vi "DMA Channel.vi"(8 "error in (no error)":errorcluster, 11 "Node Ptr":T3 format="%.0x") -> (0 "error out":errorcluster)   [LabVIEW 2020, in "FPGA Addon System Explorer.lvlib"]
uses:
  FPGA Addon System Explorer.lvlib
  <vilib>/NI VeriStand/Custom Device API/Custom Device API.lvlib
  Addon Shared/FPGA Addon Shared.lvlib
  Addon Shared/Types/FG Action.ctl
  Addon Shared/Types/Delacing Scheme.ctl
  Addon Shared/Types/DMA Acquisition Mode.ctl
  Addon Shared/Types/DMA Settings.ctl
  <vilib>/NI VeriStand/Custom Device API/Custom Device Item Ref.ctl
panel:
  in  "DMA Host Buffer":u32(ring)=5 items=["1 Second"=1, "2 Seconds"=2, "5 Seconds"=5, "10 Seconds"=10]
  out "Original Name":string
  in  "Number of Samples":u32
  in  "Mode":T1
  in  "dt":dbl format="%#_p"
  in  "Reset":bool
  in  "Apply":bool
  in  "Update Rate":u32(ring)=1 items=["1 Hz"=1, "2 Hz"=2, "5 Hz"=5, "10 Hz"=10]
  in  "Delacing Scheme":T2
  in  "Number of Channels":u8
  in  "Header 2":cluster{"Section Name":string}={"Section Name"="DMA Settings"}
  in  "SHDocVw.IWebBrowser":refnum<k7>(container)
  in  "Header":cluster{"Section Name":string}={"Section Name"="Section Settings"}
  in  "Description":string
  in  "Name":string
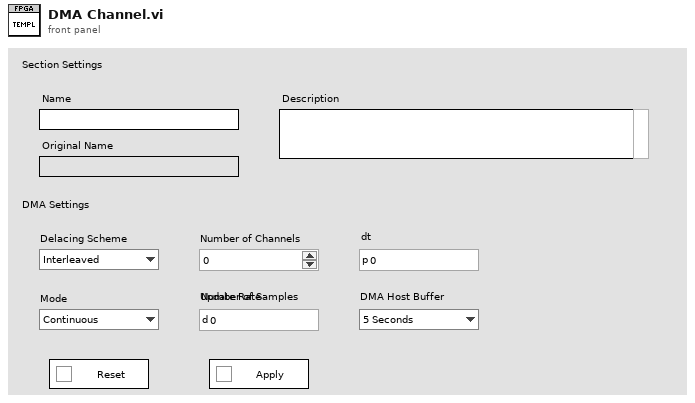
[diagram p1: front panel]
types:
  T1 = typedef "FPGA Addon Shared.lvlib/DMA Acquisition Mode.ctl" = enum8{"Continuous", "Triggered Finite"}
  T2 = typedef "FPGA Addon Shared.lvlib/Delacing Scheme.ctl" = enum8{"Interleaved", "Bitpacked"}
  T3 = typedef "Custom Device API.lvlib/Custom Device Item Ref.ctl" = u64
  T4 = typedef "FPGA Addon Shared.lvlib/FG Action.ctl" = enum8{"GET", "SET"}
  T5 = typedef "FPGA Addon Shared.lvlib/DMA Information.ctl" = cluster{"Name":string, "Data Type":T6}
  T6 = typedef "FPGA Addon Shared.lvlib/FPGA Addon Data Type.ctl" = enum8{"<Null>", "I8", "I16", "I32", "I64", "U8", "U16", "U32", "U64", "SGL", "Boolean", "Analog PWM In Settings", "Analog PWM In", "Digital PWM In Settings", "Digital PWM In", "Digital PWM Out", "Sine Out", "FXP", "FXP+/-24.5", "FXP+/-16.5", "FXP+/-32.8", "FXP+/-64.32", "FXP+/-16.7", "FXP+/-20.5", "FXP+/-27.5", "FXP+/-32.16", "FXP+16.3", "FXP+18.3", "Digital Static In", "Digital Static Out", "Digital Static In Settings", "Digital WSS Out", "Quad Encoder Settings", "Quad Encoder In", "Group"}
  T7 = typedef "Custom Device API.lvlib/Custom Device Item Info.ctl" = cluster{"Name":string, "Is Channel":bool, "GUID":string, "Is Waveform":bool}
  T8 = typedef "FPGA Addon Shared.lvlib/DMA Settings.ctl" = cluster{"Number of Channels":u8, "Delacing Scheme":T2, "Update Rate":u32, "dt":dbl, "Mode":T1, "Number of Samples":u32, "DMA Host Buffer":u32}
  T9 = typedef "Custom Device API.lvlib/Custom Device Commands.ctl" = enum16{"Default", "Item renamed", "Shutdown", "Dynamic button pressed"}
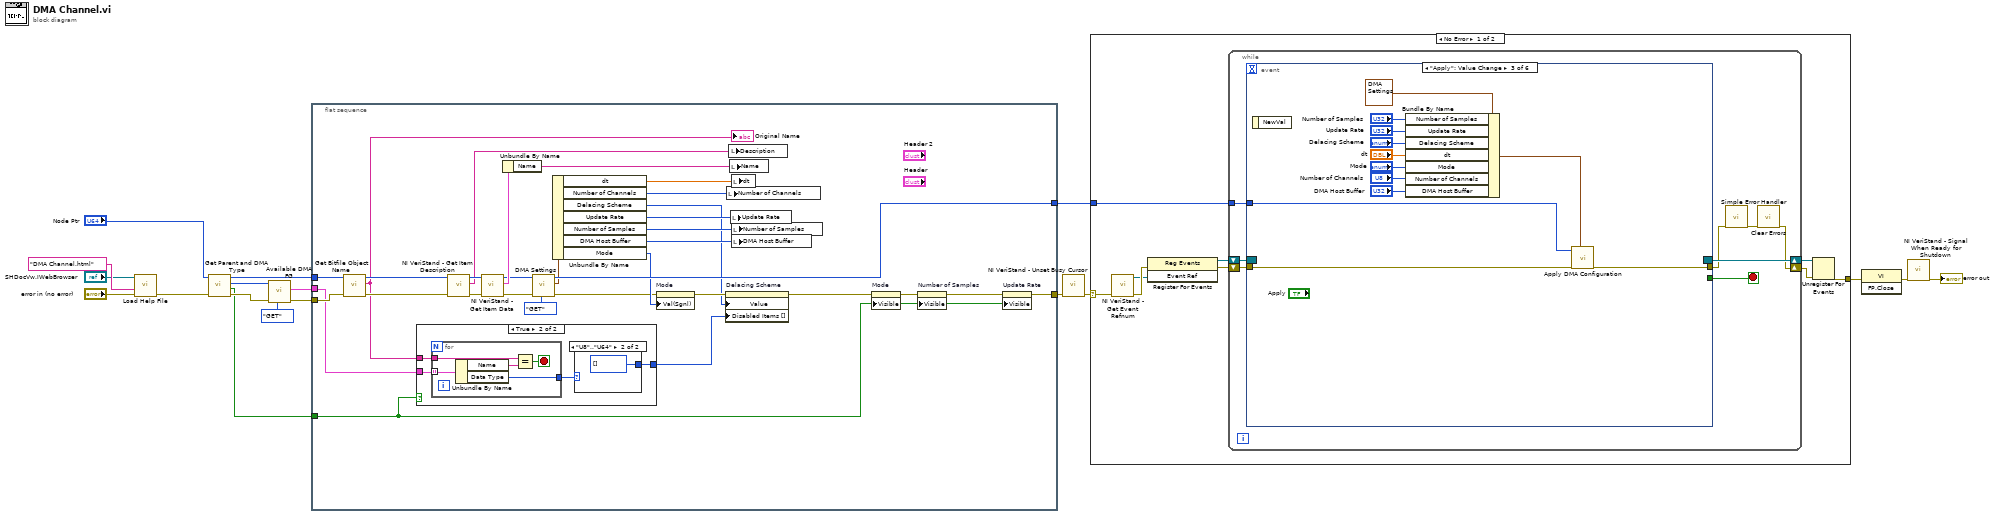
[diagram p0: block diagram]
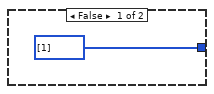
[diagram p2: hidden frame]
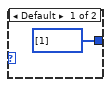
[diagram p3: hidden frame]
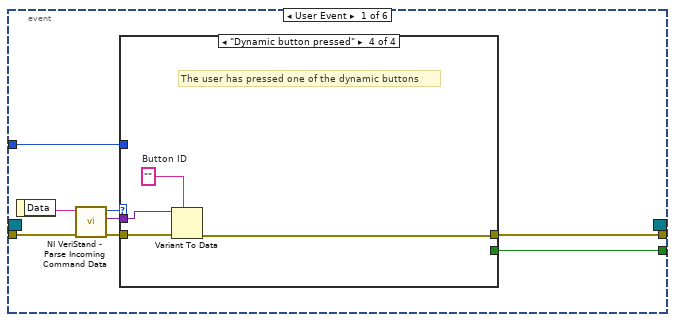
[diagram p4: hidden frame]
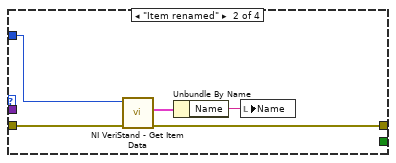
[diagram p6: hidden frame]
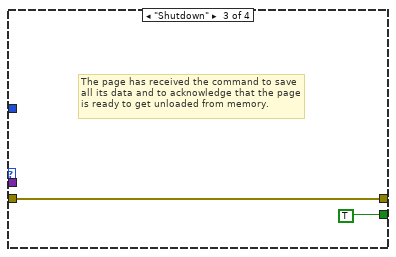
[diagram p7: hidden frame]
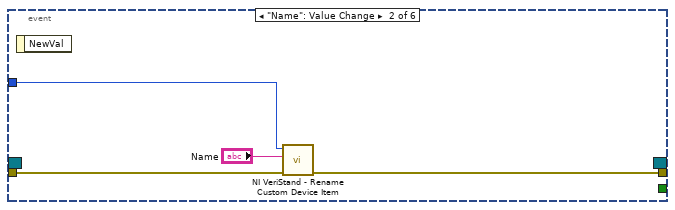
[diagram p8: hidden frame]
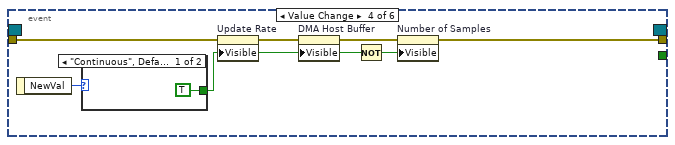
[diagram p9: hidden frame]
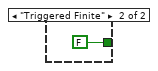
[diagram p10: hidden frame]
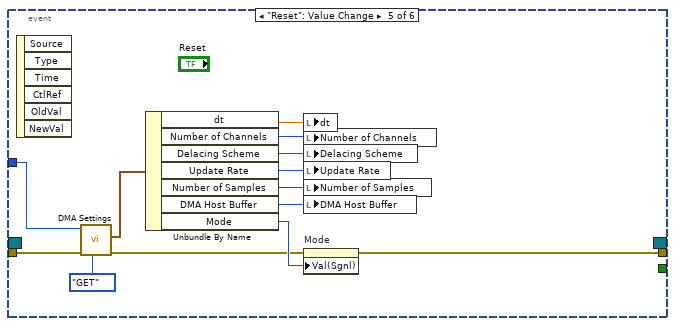
[diagram p11: hidden frame]
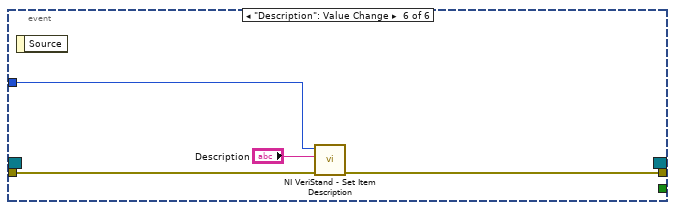
[diagram p12: hidden frame]
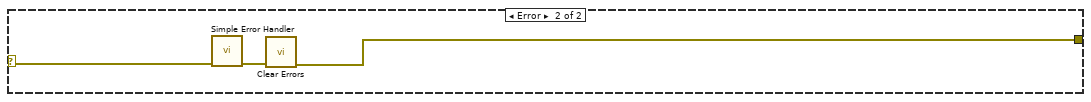
[diagram p13: hidden frame]
diagram:
  n1 = call "Load Help File.vi"("error in (no error)"="error in (no error)", "HTML File to Load"="DMA Channel.html" ("HTML File"), "SHDocVw.IWebBrowser2"="SHDocVw.IWebBrowser") -> ("error out"=w10:errorcluster)  [unwired: 8 in]
  n2 = call "Get Parent and DMA Type.vi"("error in (no error)"=w10, "Node Ptr"="Node Ptr") -> ("error out"=w6:errorcluster, "Input?"=w4:bool, "Parent Ref"=w1:T3, "Item Ref out"=w2:T3)  [unwired: 6 in]
  n3 = call "Available DMA FG.vi"("Action"=FG_Action."GET", "error in (no error)"=w6, "Item Ref"=w1) -> ("error out"=w5:errorcluster, "Available DMA"=w3:T5[])  [unwired: 6 in, 1 out]
  n4 = flat-sequence {
    tunnel: [w49] -> w14
    tunnel: w2 -> [w48]
    tunnel: [w45] -> w8
    tunnel: w5 -> [w44]
    tunnel: w4 -> [w19]
    tunnel: w3 -> [w25]
    frame #0 {
      n5 = call "Get Bitfile Object Name.vi"("error in (no error)"=w44, "Item Ref in"=w48) -> ("error out"=w29:errorcluster, "Value"=w24:string, "Item Ref out"=w28:T3)  [unwired: 7 in]
      "Original Name" <- w24
      n6 = case shown="True" w19 {
        tunnel: w25 -> [_ w54]
        tunnel: w24 -> [_ w53]
        tunnel: [i32[] [1] ("Disabled Items []") w51] -> w20
        frame False {
        }
        frame True {
          n7 = for {
            tunnel: w54 -> [w61] mode=indexing
            tunnel: w53 -> [w60]
            tunnel: [w58] -> w52
            stop <- w59 stop-if-true
            n8 = Unbundle By Name(w61) -> ("Name"=w57:string, "Data Type"=w58:T6)
            n9 = Equal?(x=w60, y=w57) -> (x = y?=w59:bool)
          }
          n10 = case shown="\"U8\"..\"U64\"" w52 {
            tunnel: [i32[] [1] ("Disabled Items []") i32[] [] ("Disabled Items []")] -> w51
            frame Default {
            }
            frame "U8".."U64" {
            }
          }
        }
      }
      n11 = call <vilib>:"NI VeriStand - Get Item Description.vi"("error in (no error)"=w29, "Item Ref in"=w28) -> ("error out"=w41:errorcluster, "Description"=w42:string, "Item Ref out"=w43:T3)  [unwired: 7 out]
      n12 = call <vilib>:"NI VeriStand - Get Item Data.vi"("error in (no error)"=w41, "Item Ref in"=w43) -> ("error out"=w38:errorcluster, "Item Info"=w40:T7, "Item Ref out"=w37:T3)  [unwired: 7 out]
      n13 = Unbundle By Name(w40) -> ("Name"=w39:string)
      n14 = call "DMA Settings.vi"("Action"=FG_Action."GET", "error in (no error)"=w38, "Item Ref"=w37) -> ("error out"=w26:errorcluster, "DMA Settings"=w35:T8, "Item Ref out"=w49:T3)  [unwired: 6 in]
      n15 = Unbundle By Name(w35) -> ("dt"=w33:dbl, "Number of Channels"=w34:u8, "Delacing Scheme"=w21:T2, "Update Rate"=w32:u32, "Number of Samples"=w31:u32, "DMA Host Buffer"=w27:u32, "Mode"=w30:T1)
      n16 = property on="Mode" class="Enum (strict)"(error in=w26, "Val(Sgnl)"=w30) -> (error out=w23:errorcluster)  [unwired: 1 in, 1 out]
      n17 = property on="Delacing Scheme" class="Enum (strict)"(error in=w23, "Value"=w21, "Disabled Items []"=w20) -> (error out=w22:errorcluster)  [unwired: 1 in, 1 out]
      n18 = local write "Number of Channels"(w34) -> ()
      n19 = local write "Description"(w42) -> ()
      n20 = local write "Name"(w39) -> ()
      n21 = local write "Update Rate"(w32) -> ()
      n22 = local write "dt"(w33) -> ()
      n23 = local write "Number of Samples"(w31) -> ()
      n24 = local write "DMA Host Buffer"(w27) -> ()
      n25 = property on="Mode" class="Enum (strict)"(error in=w22, "Visible"=w19) -> (error out=w47:errorcluster)  [unwired: 1 in, 1 out]
      n26 = property on="Number of Samples" class="DigNum (strict)"(error in=w47, "Visible"=w19) -> (error out=w46:errorcluster)  [unwired: 1 in, 1 out]
      n27 = property on="Update Rate" class="Ring (strict)"(error in=w46, "Visible"=w19) -> (error out=w45:errorcluster)  [unwired: 1 in, 1 out]
    }
  }
  n28 = call <vilib>:"NI VeriStand - Unset Busy Cursor.vi"("error in (no error)"=w8) -> ("error out"=w15:errorcluster)  [unwired: 10 out]
  n29 = case shown="No Error" w15 {
    selector: w15 -> [w62 w143]
    tunnel: [w67 w141] -> w18
    tunnel: w14 -> [w63 _]
    frame No Error {
      n30 = call <vilib>:"NI VeriStand - Get Event Refnum.vi"("error in (no error)"=w62) -> ("error out"=w70:errorcluster, "Event Ref"=w66:refnum<user-event>)  [unwired: 9 out]
      n31 = register-events(error in=w70, w66) -> (reference out=w64:refnum<event-registration>, error out=w65:errorcluster)  [unwired: 1 in]
      n32 = while {
        tunnel: w63 -> [w74]
        shift-right: [w71] -> w68
        shift-left: w65 -> [w77]
        shift-right: [w78] -> w69
        shift-left: w64 -> [w76]
        stop <- w75 stop-if-true
        n33 = event shown="[2] \"Apply\": Value Change" {
          selector: w76 -> [_ _ _ _ _ _]
          dyn-events: [_ _ _ _ _ _] -> w78
          timeout: _ -> [_ _ _ _ _ _]
          tunnel: w77 -> [w86 w102 w106 w119 w133 w139]
          tunnel: [w82 _ _ _ _ _] -> w75
          tunnel: [w81 w101 w105 w118 w125 w138] -> w73
          tunnel: w74 -> [w80 w100 w103 _ w132 w140]
          event User Event {
            n34 = event-data() -> ("Data"=w85:string)  [unwired: 1 out]
            n35 = call <vilib>:"NI VeriStand - Parse Incoming Command Data.vi"("error in (no error)"=w86, "Incoming data"=w85) -> ("error out"=w84:errorcluster, "Outgoing data"=w79:variant, "Action"=w83:T9)  [unwired: 7 out]
            n36 = case shown="\"Dynamic button pressed\"" w83 {
              tunnel: w84 -> [w87 w92 w93 w98]
              tunnel: [_ _ TRUE _] -> w82
              tunnel: [w87 w89 w93 w95] -> w81
              tunnel: w80 -> [_ w91 _ _]
              tunnel: w79 -> [_ _ _ w97]
              frame "Default", Default {
              }
              frame "Item renamed" {
                n37 = call <vilib>:"NI VeriStand - Get Item Data.vi"("error in (no error)"=w92, "Item Ref in"=w91) -> ("error out"=w89:errorcluster, "Item Info"=w90:T7)  [unwired: 8 out]
                n38 = Unbundle By Name(w90) -> ("Name"=w88:string)
                n39 = local write "Name"(w88) -> ()
              }
              frame "Shutdown" {
                # "The page has received the command to save all its data and to acknowledge that the page is ready to get unloaded from memory."
              }
              frame "Dynamic button pressed" {
                w96 = ""  # Button ID
                # "The user has pressed one of the dynamic buttons"
                n40 = Variant To Data(error in=w98, type=w96, Variant=w97) -> (error out=w95:errorcluster)  [unwired: 1 out]
              }
            }
          }
          event "Name": Value Change {
            n41 = event-data() -> ()  [unwired: 2 out]
            n42 = call <vilib>:"NI VeriStand - Rename Custom Device Item.vi"("error in (no error)"=w102, "New Name"="Name", "Item Ref in"=w100) -> ("error out"=w101:errorcluster)  [unwired: 1 in, 7 out]
          }
          event "Apply": Value Change {
            n43 = event-data() -> ()  [unwired: 2 out]
            n44 = Bundle By Name(cluster=T8 {"Number of Channels"=1, "Delacing Scheme"=enum."Interleaved", "Update Rate"=1000, "dt"=1000.0, "Mode"=enum."Continuous", "Number of Samples"=0, "DMA Host Buffer"=5} ("DMA Settings"), "Number of Samples"="Number of Samples", "Update Rate"="Update Rate", "Delacing Scheme"="Delacing Scheme", "dt"="dt", "Mode"="Mode", "Number of Channels"="Number of Channels", "DMA Host Buffer"="DMA Host Buffer") -> (w104:T8)
            n45 = call "Apply DMA Configuration.vi"("DMA Settings"=w104, "error in (no error)"=w106, "Item Ref in"=w103) -> ("error out"=w105:errorcluster)  [unwired: 8 in]
          }
          event Value Change {
            n46 = event-data() -> ("NewVal"=w120:T1)  [unwired: 1 out]
            n47 = case shown="\"Continuous\", Default" w120 {
              tunnel: [TRUE FALSE] -> w115
              frame "Continuous", Default {
              }
              frame "Triggered Finite" {
              }
            }
            n48 = property on="Update Rate" class="Ring (strict)"(error in=w119, "Visible"=w115) -> (error out=w117:errorcluster)  [unwired: 1 in, 1 out]
            n49 = property on="DMA Host Buffer" class="Ring (strict)"(error in=w117, "Visible"=w115) -> (error out=w116:errorcluster)  [unwired: 1 in, 1 out]
            n50 = Not(x=w115) -> (.not. x?=w121:bool)
            n51 = property on="Number of Samples" class="DigNum (strict)"(error in=w116, "Visible"=w121) -> (error out=w118:errorcluster)  [unwired: 1 in, 1 out]
          }
          event "Reset": Value Change {
            n52 = event-data() -> ()  [unwired: 7 out]
            n53 = call "DMA Settings.vi"("Action"=FG_Action."GET", "error in (no error)"=w133, "Item Ref"=w132) -> ("error out"=w126:errorcluster, "DMA Settings"=w131:T8)  [unwired: 6 in, 1 out]
            n54 = Unbundle By Name(w131) -> ("dt"=w129:dbl, "Number of Channels"=w130:u8, "Delacing Scheme"=w135:T2, "Update Rate"=w136:u32, "Number of Samples"=w127:u32, "DMA Host Buffer"=w124:u32, "Mode"=w128:T1)
            n55 = local write "dt"(w129) -> ()
            n56 = local write "Number of Channels"(w130) -> ()
            n57 = local write "Delacing Scheme"(w135) -> ()
            n58 = local write "Update Rate"(w136) -> ()
            n59 = local write "Number of Samples"(w127) -> ()
            n60 = local write "DMA Host Buffer"(w124) -> ()
            n61 = property on="Mode" class="Enum (strict)"(error in=w126, "Val(Sgnl)"=w128) -> (error out=w125:errorcluster)  [unwired: 1 in, 1 out]
          }
          event "Description": Value Change {
            n62 = event-data() -> ()  [unwired: 2 out]
            n63 = call <vilib>:"NI VeriStand - Set Item Description.vi"("error in (no error)"=w139, "Description"="Description", "Item Ref in"=w140) -> ("error out"=w138:errorcluster)  [unwired: 8 out]
          }
        }
        n64 = call <vilib>:"Simple Error Handler.vi"("error in (no error)"=w73) -> ("error out"=w72:errorcluster)  [unwired: 1 in, 7 out]
        n65 = call <vilib>:"Clear Errors.vi"("error in (no error)"=w72) -> ("error out"=w71:errorcluster)  [unwired: 1 in, 5 out]
      }
      n66 = Unregister For Events(event registration refnum=w69, error in=w68) -> (error out=w67:errorcluster)
    }
    frame Error {
      n67 = call <vilib>:"Simple Error Handler.vi"("error in (no error)"=w143) -> ("error out"=w142:errorcluster)  [unwired: 1 in, 7 out]
      n68 = call <vilib>:"Clear Errors.vi"("error in (no error)"=w142) -> ("error out"=w141:errorcluster)  [unwired: 1 in, 5 out]
    }
  }
  n69 = invoke class="VI" method="FP.Close"(error in=w18) -> (error out=w17:errorcluster)  [unwired: 2 in, 2 out]
  n70 = call <vilib>:"NI VeriStand - Signal When Ready for Shutdown.vi"("error in (no error)"=w17) -> ("error out"=→"error out":errorcluster)  [unwired: 10 out]
